vi "VIH Constant - Temporal Folder.vi"(11 "append path":path) -> (3 "Temporal folder":path)   [LabVIEW 2014]
doc: "::: VI Helpeks :::\nCopyright (c) 2000-2026 Konstantin Shifershteyn. All rights reserved."
panel:
  # "VI Helpeks\nCopyright (c) 2012-2026 Konstantin Shifershteyn"
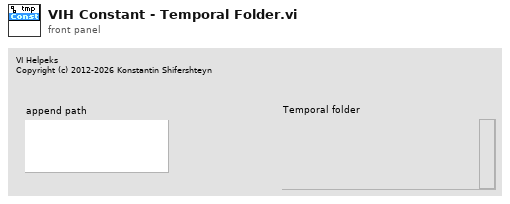
[diagram p1: front panel]
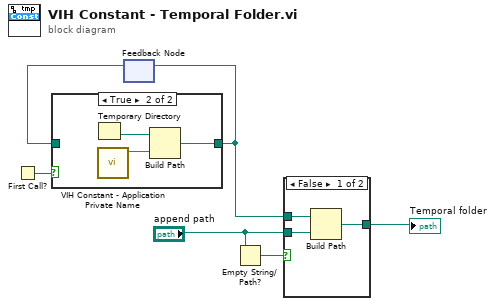
[diagram p0: block diagram]
diagram:
  n1 = First Call?() -> (First Call?: T/F=w3:bool)
  n2 = feedback #1() -> (w1:path)  [unwired: 1 in]
  n3 = case shown="True" w3 {
    tunnel: [w7 w8] -> w2
    tunnel: w1 -> [w7 _]
    frame False {
    }
    frame True {
      n4 = Temporary Directory() -> (w10:path)
      n5 = call "VIH Constant - Application Private Name.vi"() -> ("Name out"=w9:string)  [unwired: 11 in]
      n6 = Build Path(base path=w10, name or relative path=w9) -> (appended path=w8:path)
    }
  }
  n7 = feedback-in #1(w2) -> ()
  n8 = Empty String/Path?(string/path="append path") -> (empty?=w4:bool)
  n9 = case shown="False" w4 {
    tunnel: w2 -> [w13 w14]
    tunnel: "append path" -> [w12 _]
    tunnel: [w11 w14] -> w5
    frame False {
      n10 = Build Path(base path=w13, name or relative path=w12) -> (appended path=w11:path)
    }
    frame True {
    }
  }
  "Temporal folder" <- w5
